vi "Read event callback refnum.vi"(8 "error in (no error)":errorcluster, 11 "ToastService in":refnum<class "ToastService.lvclass">) -> (0 "error out":errorcluster, 2 "event callback refnum":refnum<k27>, 3 "ToastService out":refnum<class "ToastService.lvclass">)   [LabVIEW 2026, in "ToastNotification.lvlib" / "ToastService.lvclass"]
doc: "Native data-member read accessor for the service event callback refnum. The output is a borrowed alias of the stored registration. Does not register, unregister or duplicate an event subscription. The service cleanup owns unregistration. Pass the class and error through."
uses:
  ToastService.lvclass
  ToastService.lvclass/ToastService.ctl
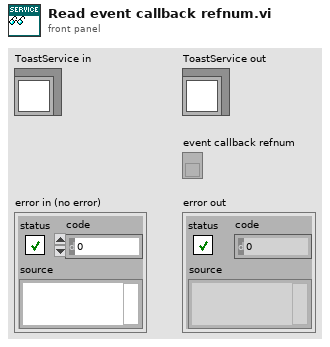
[diagram p1: front panel]
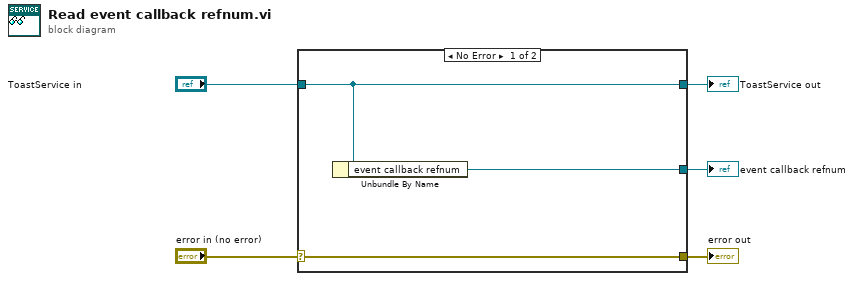
[diagram p0: block diagram]
diagram:
  n1 = case shown="No Error" "error in (no error)" {
    selector: "error in (no error)" -> [w8 w9]
    tunnel: [w8 w9] -> w4
    tunnel: [w7 w10] -> w2
    tunnel: "ToastService in" -> [w7 w10]
    tunnel: [w6 _] -> w1
    frame No Error {
      n2 = Unbundle By Name(w7) -> ("event callback refnum"=w6:refnum<k27>)
    }
    frame Error {
    }
  }
  "error out" <- w4
  "ToastService out" <- w2
  "event callback refnum" <- w1
